vi "Host Image Acquisition Module.vi"(8 "error in":errorcluster, 11 "Operation":T3) -> (0 "error out":errorcluster, 1 "Image Acquired":bool, 2 "Acq In Progress":bool, 3 "Image":T2(plugin-control), 4 "Frames To Acquire":u32, 5 "Num Frames read":u32)   [LabVIEW 2013]
uses:
  Host Image Acquisition Module Enum.ctl
  Acquisition Settings Cluster.ctl
  Image Acquisition Settings FG Enum.ctl
  System Status/Status FG Enum.ctl
  Image Processing/Mask ROI FG Enum.ctl
  <vilib>/rvi/interface/common/niFpgaWaitOnOcc.vi
  <vilib>/FPGAPlugInAG/PCIe-1473R/niLvFpga_Reset_PCIe-1473R.vi
  <vilib>/Utility/error.llb/Error Cluster From Error Code.vi
  <vilib>/rvi/errors/niLvFpgaAdjustHostInterfaceError.vi
  <vilib>/FPGAPlugInAG/PCIe-1473R/niLvFpga_Run_PCIe-1473R.vi
  Globals/Average Sector Data.vi
  <vilib>/FPGAPlugInAG/PCIe-1473R/niLvFpga_Close_PCIe-1473R.vi
  <vilib>/rvi/interface/nirviMethod/nirviMethod.xnode
  FGs/FPGA_Reference.ctl
  FPGA Bitfiles/Simulation_WBA.lvbitx
  <vilib>/rvi/interface/nirviReadWriteControl/nirviReadWriteControl.xnode
  Common/CL Configuration.ctl
  Common/CL Signal Mapping.ctl
  FPGA/Sector/Accumulate/Sector Parameter Cluster.ctl
  <vilib>/rvi/interface/nirviCloseFPGA/nirviCloseFPGA.xnode
  Common/Timing/Timing Lib.lvlib
  NiFpgaLv.dll
  <vilib>/rvi/errors/niLvFpgaMergeErrorWithErrorCode.vi
  <vilib>/FPGAPlugInAG/PCIe-1473R/niLvFpga_ReadFifo_PCIe-1473R.vi
  <vilib>/FPGAPlugInAG/PCIe-1473R/niLvFpga_ConfigureFifo_PCIe-1473R.vi
  <vilib>/FPGAPlugInAG/PCIe-1473R/niLvFpga_StartFifo_PCIe-1473R.vi
panel:
  out "Actual Depth":u32
  out "Target Sim TO":bool
  out "Cam Data Timeout":bool
  out "Sector FIFO Timeout":bool
  out "Host DMA Timeout":bool
  out "Number of Elements to Write Host DMA":u32
  out "Number of Elements to Read Cam Data":u32
  out "Image Data":u64[](array[numeric])
  out "Elements Remaining":u32
  out "Words per image":u32
  out "DMA Words per Image":u32
  out "Acquire":bool
  in  "Acquisition Settings Cluster":T1={"Image Width"=1200, "Image Height"=788, "Frames To Acquire"=0, "Signal Mapping"=enum."Standard", "DMA Buffer Size\n(In Images)"=2200} {"Image Height" max=65535; "Image Width" max=65535 step=40}
  out "Buffer Size":u32
  out "Acq'd Frame Width":u32=2040
  out "DMA Write Timeout":bool
  in  "Start Serial Server":bool
  out "Frames Acq'd":u32=1
  out "Acq'd Frame Height":u32=1088
  out "Initialized":bool
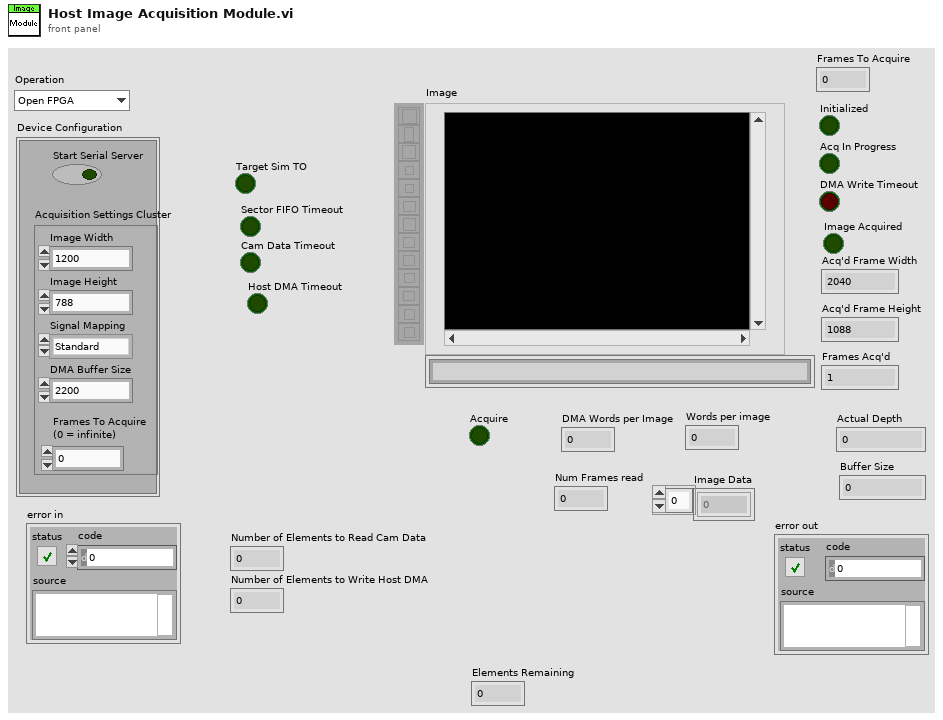
[diagram p1: front panel]
types:
  T1 = typedef "Acquisition Settings Cluster.ctl" = cluster{"Image Width":u32, "Image Height":u32, "Frames To Acquire":u32, "Signal Mapping":enum8{"Standard", "Basler 10-tap", "Vosskühler 10-tap"}, "DMA Buffer Size\n(In Images)":u32}
  T2 = typedef "IMAQ Image.ctl" = refnum<image>
  T3 = typedef "Host Image Acquisition Module Enum.ctl" = enum16{"Open FPGA", "Initialize DMA FIFO", "Load Sim Images", "Initialize Acquisition", "Update Sector Parameters", "Start Acquisition", "Aquire Image", "Read Averages", "Cancel Acquisition", "Close FPGA"}
  T4 = enum8{"Standard", "Basler 10-tap", "Vosskühler 10-tap"}
  T5 = typedef "Image Acquisition Settings FG Enum.ctl" = enum16{"Read", "Write"}
  T6 = typedef "Status FG Enum.ctl" = enum16{"Reset", "Read", "Write"}
  T7 = typedef "Mask ROI FG Enum.ctl" = enum16{"Read", "Write", "Enable Background", "Disable Background"}
  T8 = enum16{"big-endian, network order", "native, host order", "little-endian"}
  T9 = typedef "FPGA_Reference.ctl" = refnum<k20>
  T10 = typedef "Mask ROI Cluster.ctl" = cluster{"left annulus":T11, "right annulus":T11, "Threshold Range":cluster{"Lower value":dbl, "Upper value":dbl}, "[Avg BG]":u8[], "Number of Sectors":u8, "Left ROI":T12, "Right ROI":T12, "Left Start Angle Duty Cycle":fxp<+,8,0>, "Left End Angle Duty Cycle":fxp<+,8,0>, "Right End Angle Duty Cycle":fxp<+,8,0>, "Right Start Angle Duty Cycle":fxp<+,8,0>, "[Sector ROIs]":T12[]}
  T11 = typedef "IMAQ Circle" = cluster{"Center X":i32, "Center Y":i32, "Inner Radius":i32, "Outer Radius":i32, "Start Angle":dbl, "End Angle":dbl}
  T12 = typedef "ROI Descriptor" = cluster{"Global Rectangle":i32[], "Contours":cluster{"ID":enum32{"External", "Internal"}, "Type":u32, "Coordinates":i32[]}[]}
  T13 = typedef "Sector Parameter Cluster.ctl" = cluster{"Start Angle":fxp<+/-,17,2>, "End Angle":fxp<+/-,17,2>, "Inner Radius":u16, "Outter Radius":u16, "Hinge X":u16, "Hinge Y":u16, "NumWingSectors":u8}
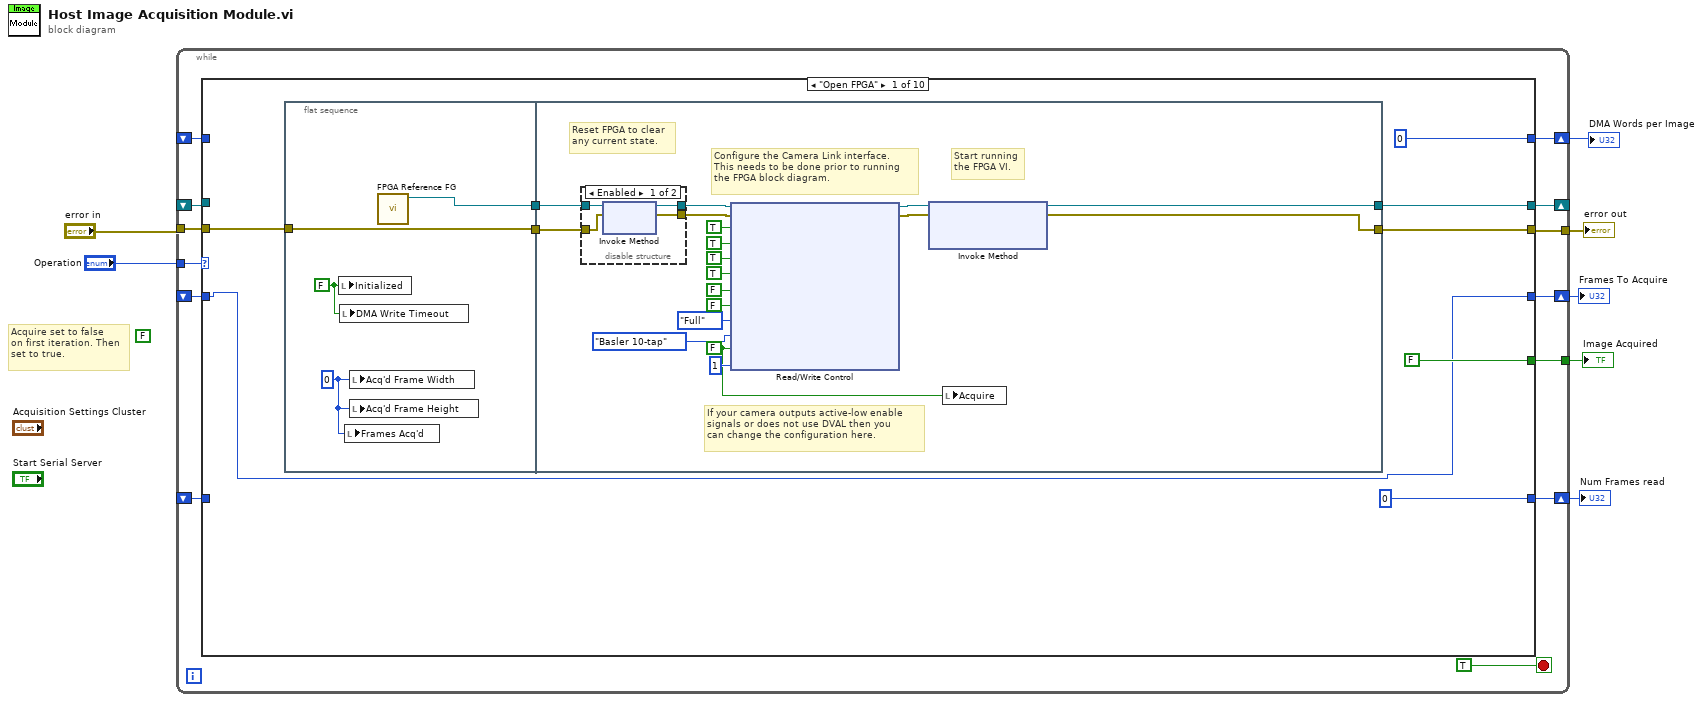
[diagram p0: block diagram]
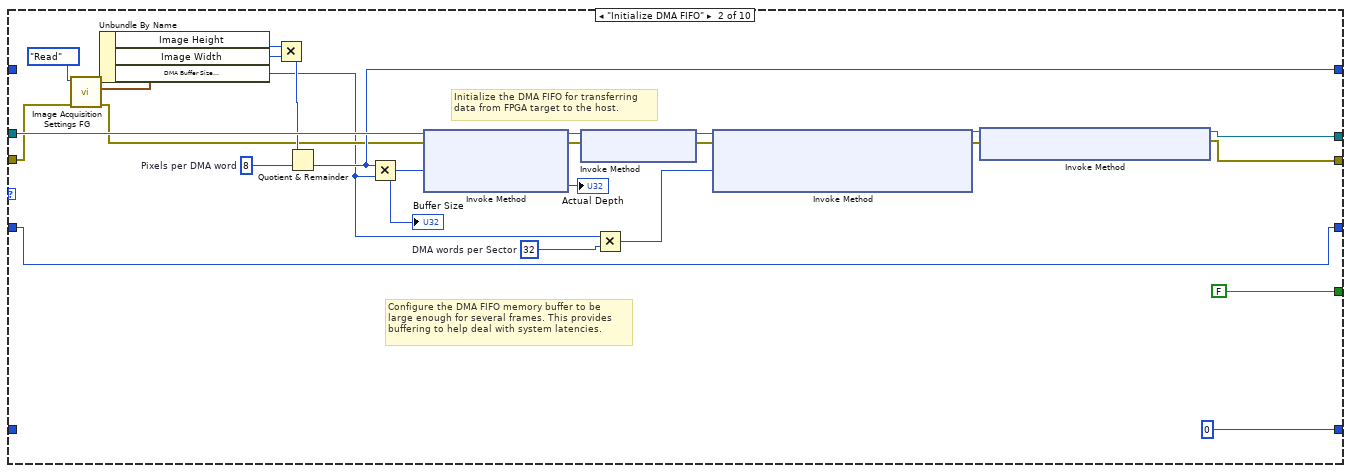
[diagram p3: hidden frame]
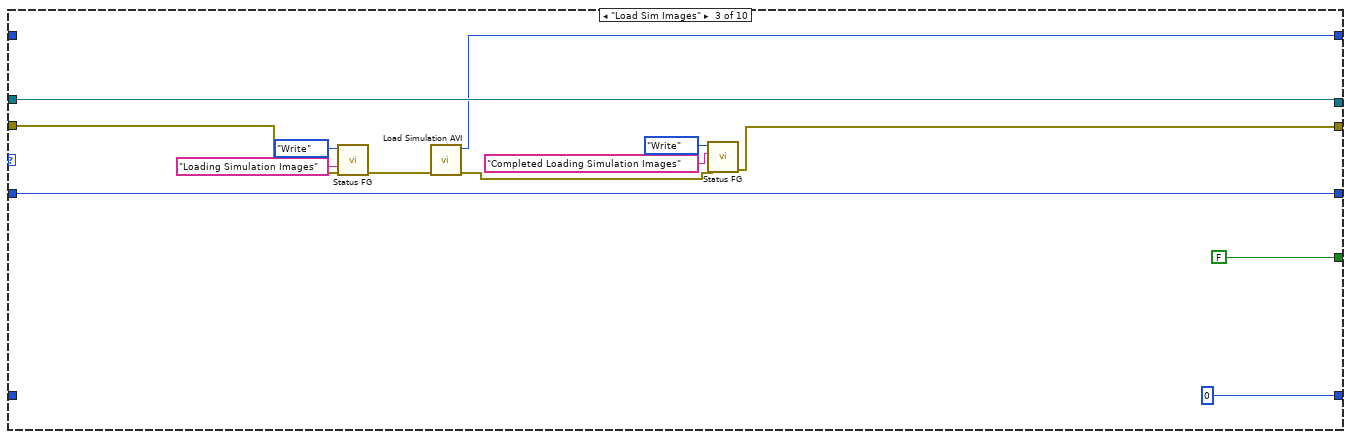
[diagram p4: hidden frame]
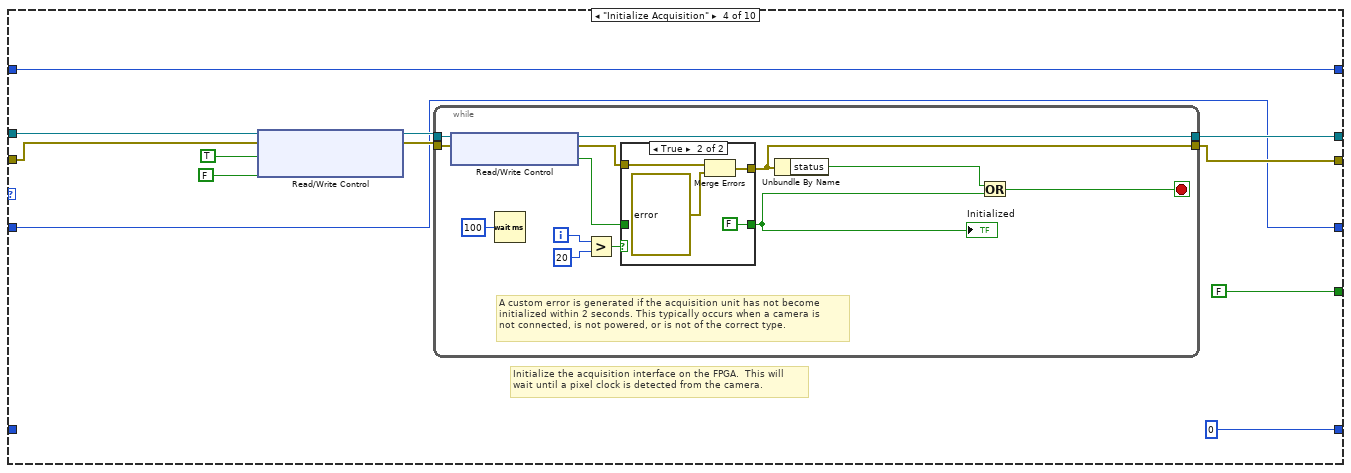
[diagram p5: hidden frame]
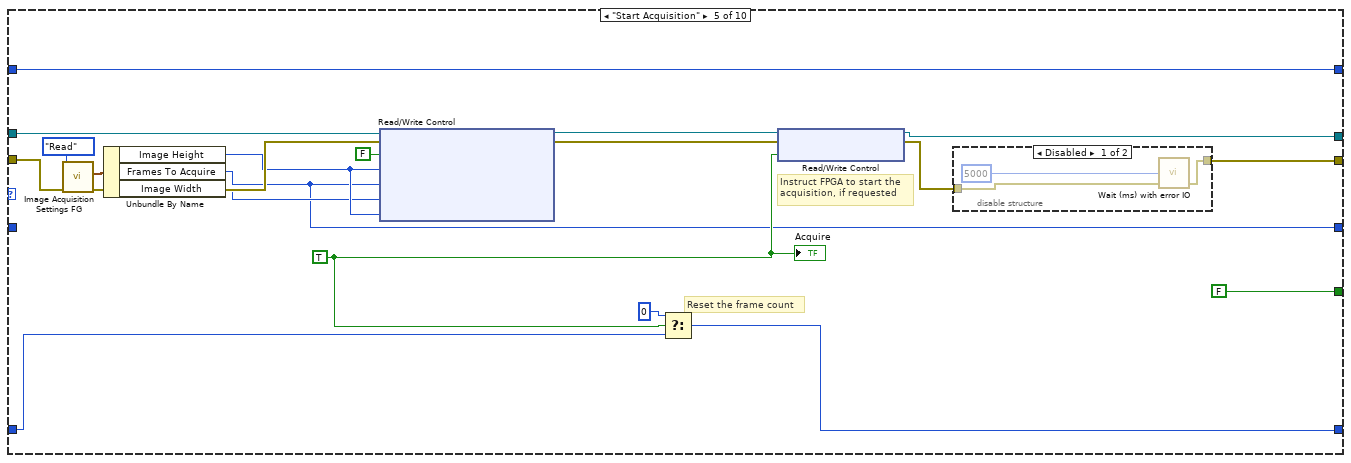
[diagram p7: hidden frame]
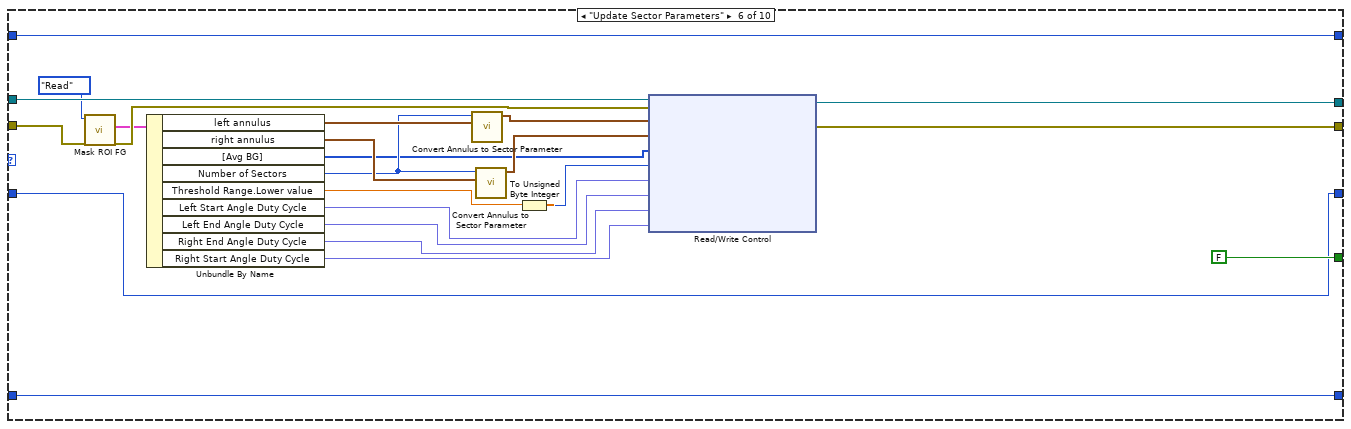
[diagram p9: hidden frame]
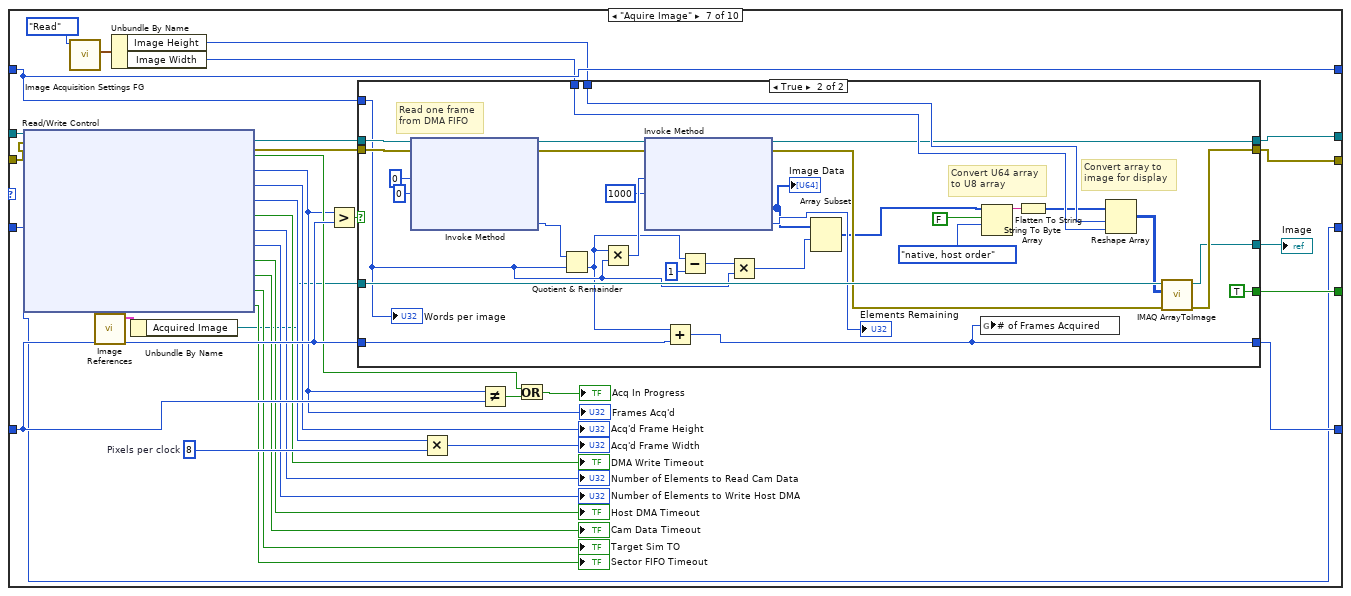
[diagram p10: hidden frame]
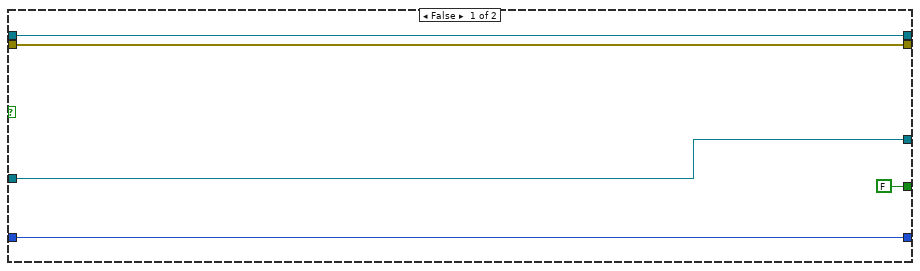
[diagram p11: hidden frame]
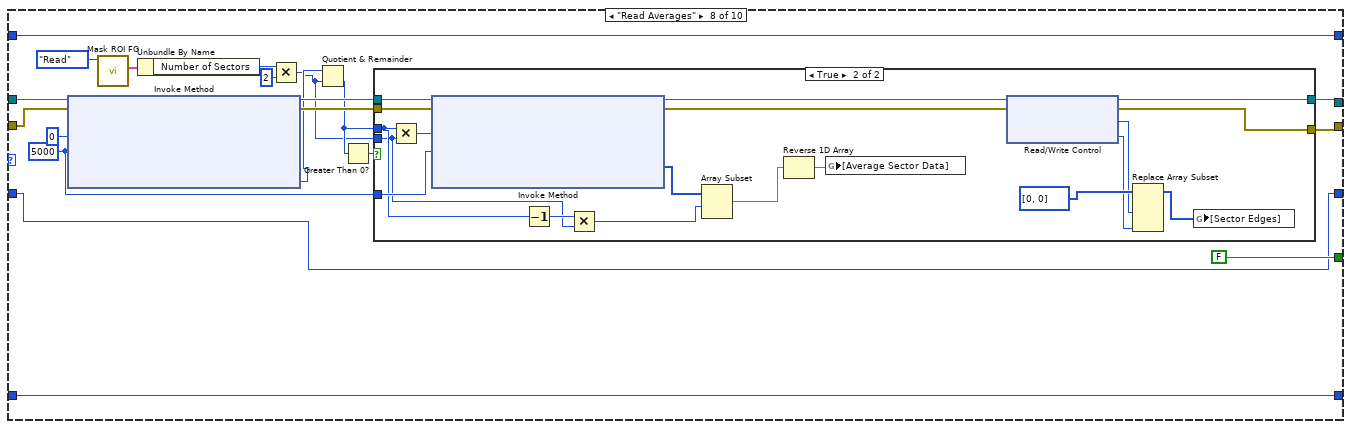
[diagram p12: hidden frame]
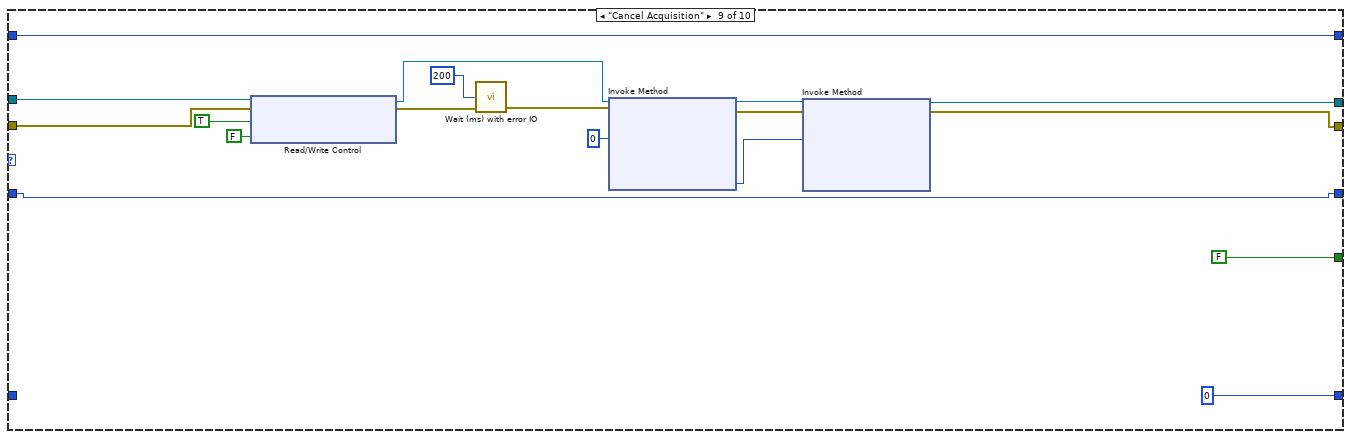
[diagram p14: hidden frame]
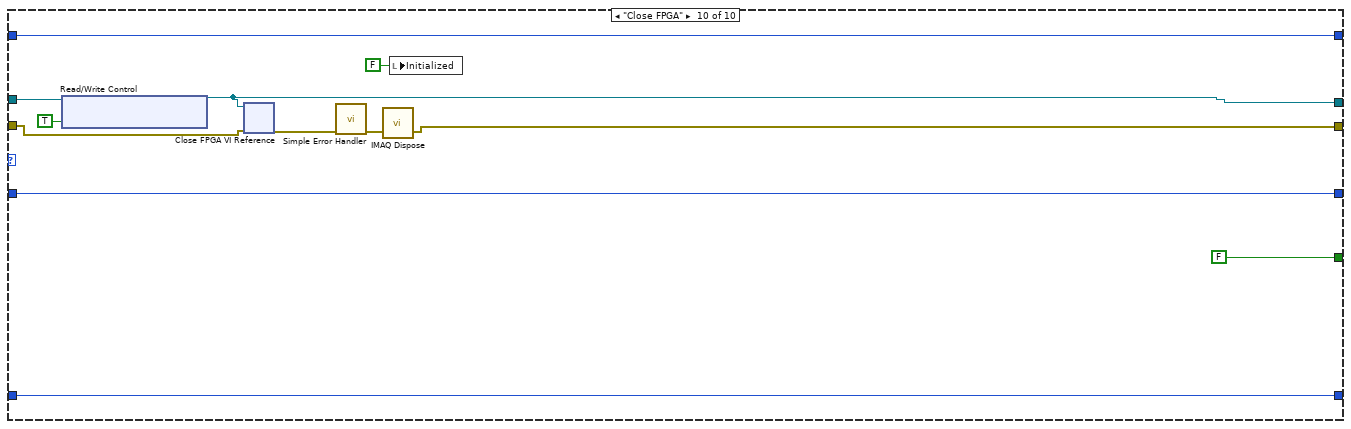
[diagram p15: hidden frame]
diagram:
  (unwired) FALSE ("Acquire")
  # "Acquire set to false\non first iteration. Then\nset to true."
  n1 = while {
    shift-right: [w19] -> _
    shift-left: _ -> [w15]
    tunnel: "error in" -> [w18]
    tunnel: "Operation" -> [w17]
    tunnel: [w16] -> w5
    shift-right: [w14] -> w4
    shift-left: _ -> [w13]
    shift-right: [w12] -> w3
    shift-left: _ -> [w11]
    tunnel: [w10] -> w2
    shift-right: [w9] -> w1
    shift-left: _ -> [w8]
    stop <- TRUE stop-if-true
    n2 = case shown="\"Open FPGA\"" w17 {
      tunnel: w18 -> [w29 w80 w92 w103 w146 w172 w203 w259 w303 w311]
      tunnel: [w28 w79 w95 w107 w142 w170 w207 w264 w289 w312] -> w19
      tunnel: [w27 w59 w91 w104 w141 w171 w206 w260 w288 w316] -> w16
      tunnel: w15 -> [_ w83 w95 w108 w147 w174 w208 w265 w304 w313]
      tunnel: [u32 0 w82 w94 w106 w143 w173 w204 w263 w302 w314] -> w14
      tunnel: w13 -> [_ _ _ w106 w143 w173 w204 w263 w302 w314]
      tunnel: [u32 0 u32 0 u32 0 u32 0 w144 w169 w205 w262 u32 0 w315] -> w12
      tunnel: w11 -> [_ _ _ _ w145 w169 w202 w262 _ w315]
      tunnel: [FALSE ("Image Acquired") FALSE ("Image Acquired") FALSE ("Image Acquired") FALSE ("Image Acquired") FALSE ("Image Acquired") FALSE ("Image Acquired") w201 FALSE ("Image Acquired") FALSE ("Image Acquired") FALSE ("Image Acquired")] -> w10
      tunnel: [w21 w58 w84 w97 w128 w152 w175 w246 w287 w305] -> w9
      tunnel: w8 -> [w21 w58 w84 w97 _ w152 w175 w246 w287 w305]
      frame "Open FPGA" {
        n3 = flat-sequence {
          tunnel: w29 -> [w30]
          tunnel: [w31] -> w26
          tunnel: [w30] -> w25
          tunnel: [w48] -> w27
          tunnel: [w49] -> w28
          tunnel: w26 -> [w51]
          tunnel: w25 -> [w50]
          frame #0 {
            w32 = u32 0 ("Acq'd Frame Width")
            w33 = FALSE ("Initialized")
            n4 = local write "Initialized"(w33) -> ()
            n5 = local write "DMA Write Timeout"(w33) -> ()
            n6 = local write "Frames Acq'd"(w32) -> ()
            n7 = local write "Acq'd Frame Width"(w32) -> ()
            n8 = local write "Acq'd Frame Height"(w32) -> ()
            n9 = call "FPGA Reference FG.vi"() -> ("FPGA VI Reference Out"=w31:T9)  [unwired: 11 in]
          }
          frame #1 {
            w34 = FALSE ("Acq Control.Acquire")
            # "If your camera outputs active-low enable\nsignals or does not use DVAL then you \ncan change the configuration here."
            # "Start running\nthe FPGA VI."
            # "Reset FPGA to clear\nany current state."
            # "Configure the Camera Link interface.\nThis needs to be done prior to running\nthe FPGA block diagram."
            n10 = disable-structure shown="Enabled" {
              disable-tunnel: [w55 w57] -> w41
              disable-tunnel: [w54 w56] -> w39
              disable-tunnel: w51 -> [w53 w57]
              disable-tunnel: w50 -> [w52 w56]
              frame Enabled {
                n11 = xnode "Invoke Method"("FPGA VI Reference In"=w53, "error in"=w52) -> ("FPGA VI Reference Out"=w55:T9, "error out"=w54:errorcluster)
              }
              frame Disabled {
              }
            }
            n12 = xnode "Read/Write Control"("FPGA VI Reference In"=w41, "error in"=w39, "CL Config.FVAL Active High"=TRUE ("IO Module Config.CL FVAL Active High"), "CL Config.LVAL Active High"=TRUE ("IO Module Config.CL LVAL Active High"), "CL Config.DVAL Active High"=TRUE ("IO Module Config.CL DVAL Active High"), "CL Config.Spare Active High"=TRUE ("IO Module Config.CL Spare Active High"), "CL Config.Line Scan"=FALSE, "Acq Control.Ignore DVAL"=FALSE ("CL Config.Line Scan"), "CL Config.Configuration"=enum8{"Base", "Medium", "Full"}."Full", "CL Config.Signal Mapping"=T4."Basler 10-tap", "Acq Control.Acquire"=w34, "# of Frames to Average"=u8 1) -> ("FPGA VI Reference Out"=w38:T9, "error out"=w40:errorcluster)
            n13 = xnode "Invoke Method"("FPGA VI Reference In"=w38, "error in"=w40) -> ("FPGA VI Reference Out"=w49:T9, "error out"=w48:errorcluster)  [unwired: 1 in]
            n14 = local write "Acquire"(w34) -> ()
          }
        }
      }
      frame "Initialize DMA FIFO" {
        w62 = u32 32  # DMA words per Sector
        w74 = u32 8  # Pixels per DMA word
        # "Configure the DMA FIFO memory buffer to be\nlarge enough for several frames. This provides\nbuffering to help deal with system latencies."
        # "Initialize the DMA FIFO for transferring\ndata from FPGA target to the host."
        n15 = call "Image Acquisition Settings FG.vi"("error in (no error)"=w80, "Operation"=Image_Acquisition_Settings_FG_Enum."Read") -> ("error out"=w68:errorcluster, "Acquisition Settings Out"=w71:T1)  [unwired: 8 in]
        n16 = Unbundle By Name(w71) -> ("Image Height"=w70:u32, "Image Width"=w69:u32, "DMA Buffer Size\n(In Images)"=w61:u32)
        n17 = Multiply(x=w70, y=w69) -> (x*y=w73:u32)
        n18 = Quotient & Remainder(x=w73, y=w74) -> (floor(x/y)=w82:u32)  [unwired: 1 out]
        n19 = Multiply(x=w82, y=w61) -> (x*y=w75:u32)
        "Buffer Size" <- w75
        n20 = xnode "Invoke Method"("FPGA VI Reference In"=w83, "error in"=w68, "Requested Depth"=w75) -> ("FPGA VI Reference Out"=w77:T9, "error out"=w76:errorcluster, "Actual Depth"=→"Actual Depth":u32)
        n21 = xnode "Invoke Method"("FPGA VI Reference In"=w77, "error in"=w76) -> ("FPGA VI Reference Out"=w67:T9, "error out"=w65:errorcluster)
        n22 = Multiply(x=w61, y=w62) -> (x*y=w60:u32)
        n23 = xnode "Invoke Method"("FPGA VI Reference In"=w67, "error in"=w65, "Requested Depth"=w60) -> ("FPGA VI Reference Out"=w64:T9, "error out"=w63:errorcluster)  [unwired: 1 out]
        n24 = xnode "Invoke Method"("FPGA VI Reference In"=w64, "error in"=w63) -> ("FPGA VI Reference Out"=w79:T9, "error out"=w59:errorcluster)
      }
      frame "Load Sim Images" {
        n25 = call "Status FG.vi"("error in (no error)"=w92, "Status In"="Loading Simulation Images", "Operation"=Status_FG_Enum."Write") -> ("error out"=w90:errorcluster)  [unwired: 7 in, 1 out]
        n26 = call "Load Simulation AVI.vi"("error in (no error)"=w90) -> ("error out"=w86:errorcluster, "Words per image"=w94:u32)  [unwired: 9 in]
        n27 = call "Status FG.vi"("error in (no error)"=w86, "Status In"="Completed Loading Simulation Images", "Operation"=Status_FG_Enum."Write") -> ("error out"=w91:errorcluster)  [unwired: 7 in, 1 out]
      }
      frame "Initialize Acquisition" {
        # "Initialize the acquisition interface on the FPGA.  This will\nwait until a pixel clock is detected from the camera."
        n28 = xnode "Read/Write Control"("FPGA VI Reference In"=w108, "error in"=w103, "Acq Control.Initialize"=TRUE ("Arm Acquisition"), "Acq Control.Cancel Acq"=FALSE) -> ("FPGA VI Reference Out"=w101:T9, "error out"=w100:errorcluster)
        n29 = while {
          tunnel: w101 -> [w117]
          tunnel: w100 -> [w116]
          tunnel: [w115] -> w107
          tunnel: [w118] -> w104
          i -> [w111]
          stop <- w121 stop-if-true
          # "A custom error is generated if the acquisition unit has not become\ninitialized within 2 seconds. This typically occurs when a camera is\nnot connected, is not powered, or is not of the correct type."
          n30 = xnode "Read/Write Control"("FPGA VI Reference In"=w117, "error in"=w116) -> ("FPGA VI Reference Out"=w115:T9, "error out"=w114:errorcluster, "Acq Status.Initialized"=w113:bool)
          n31 = Wait (ms)(milliseconds to wait=u32 100) -> ()  [unwired: 1 out]
          n32 = Greater?(x=w111, y=20) -> (0:w112:bool)
          n33 = case shown="True" w112 {
            tunnel: [w123 FALSE] -> w109
            tunnel: w113 -> [w123 _]
            tunnel: w114 -> [w122 w125]
            tunnel: [w122 w127] -> w118
            frame False {
            }
            frame True {
              n34 = Merge Errors(w125, errorcluster {"status"=TRUE, "code"=-8999, "source"="Acquisition Initialization: This error typically occurs when a camera is not properly connected, is not powered, or is not of the correct type."} ("error in")) -> (w127:errorcluster)
            }
          }
          "Initialized" <- w109
          n35 = Unbundle By Name(w118) -> ("status"=w120:bool)
          n36 = Or(x=w120, y=w109) -> (x .or. y?=w121:bool)
        }
      }
      frame "Start Acquisition" {
        w136 = TRUE ("Acquire")
        # "Reset the frame count"
        # "Instruct FPGA to start the\nacquisition, if requested"
        n37 = call "Image Acquisition Settings FG.vi"("error in (no error)"=w146, "Operation"=Image_Acquisition_Settings_FG_Enum."Read") -> ("error out"=w135:errorcluster, "Acquisition Settings Out"=w139:T1)  [unwired: 8 in]
        n38 = Unbundle By Name(w139) -> ("Image Height"=w130:u32, "Frames To Acquire"=w128:u32, "Image Width"=w129:u32)
        n39 = xnode "Read/Write Control"("FPGA VI Reference In"=w147, "error in"=w135, "Acq Control.Cancel Acq"=FALSE, "Acq Control.Line Scan Height"=w130, "Acq Control.Frames To Acq"=w128, "X Resolution"=w129, "Y Resolution"=w130) -> ("FPGA VI Reference Out"=w131:T9, "error out"=w132:errorcluster)
        n40 = Select(t=u32 0, s=w136, f=w145) -> (s? t:f=w144:u32)
        n41 = xnode "Read/Write Control"("FPGA VI Reference In"=w131, "error in"=w132, "Acq Control.Acquire"=w136) -> ("FPGA VI Reference Out"=w142:T9, "error out"=w133:errorcluster)
        n42 = disable-structure shown="Disabled" {
          disable-tunnel: w133 -> [w149 w151]
          disable-tunnel: [w148 w151] -> w141
          frame Disabled {
            n43 = call "Wait (ms) with error IO.vi"("error in (no error)"=w149, "milliseconds to wait"=u32 5000) -> ("error out"=w148:errorcluster)  [unwired: 3 in]
          }
          frame Enabled {
          }
        }
        "Acquire" <- w136
      }
      frame "Update Sector Parameters" {
        n44 = call "Mask ROI FG.vi"("error in (no error)"=w172, "Operation"=Mask_ROI_FG_Enum."Read") -> ("error out"=w167:errorcluster, "Mask ROI Out"=w165:T10)  [unwired: 8 in]
        n45 = Unbundle By Name(w165) -> ("left annulus"=w164:T11, "right annulus"=w162:T11, "[Avg BG]"=w159:u8[], "Number of Sectors"=w161:u8, "Threshold Range.Lower value"=w158:dbl, "Left Start Angle Duty Cycle"=w156:fxp<+,8,0>, "Left End Angle Duty Cycle"=w155:fxp<+,8,0>, "Right End Angle Duty Cycle"=w154:fxp<+,8,0>, "Right Start Angle Duty Cycle"=w153:fxp<+,8,0>)
        n46 = call "Convert Annulus to Sector Parameter.vi"("Annulus"=w164, "NumWingSectors"=w161) -> ("Sector Parameter"=w163:T13)  [unwired: 9 in]
        n47 = call "Convert Annulus to Sector Parameter.vi"("Annulus"=w162, "NumWingSectors"=w161) -> ("Sector Parameter"=w160:T13)  [unwired: 9 in]
        n48 = To Unsigned Byte Integer(number=w158) -> (unsigned 8bit integer=w157:u8)
        n49 = xnode "Read/Write Control"("FPGA VI Reference In"=w174, "error in"=w167, "Sector Parameters Left"=w163, "Sector Parameters Right"=w160, "[Average BG Intensity]"=w159, "Sector Threshold"=w157, "Left Start Angle Duty Cycle"=w156, "Left End Angle Duty Cycle"=w155, "Right End Angle Duty Cycle"=w154, "Right Start Angle Duty Cycle"=w153) -> ("FPGA VI Reference Out"=w170:T9, "error out"=w171:errorcluster)
      }
      frame "Aquire Image" {
        w196 = u32 8  # Pixels per clock
        n50 = xnode "Read/Write Control"("FPGA VI Reference In"=w208, "error in"=w203) -> ("FPGA VI Reference Out"=w200:T9, "error out"=w199:errorcluster, "Acq Status.Acq In Progress"=w188:bool, "Acq Status.Frames Acq'd"=w187:u32, "Acq Status.Lines Per Frame"=→"Acq'd Frame Height":u32, "Acq Status.Clocks Per Line"=w195:u32, "Acq Status.DMA Write Timeout"=→"DMA Write Timeout":bool, "Number of Elements to Read Cam Data"=→"Number of Elements to Read Cam Data":u32, "Number of Elements to Write Host DMA"=→"Number of Elements to Write Host DMA":u32, "Host DMA Timeout"=→"Host DMA Timeout":bool, "Cam Data Timeout"=→"Cam Data Timeout":bool, "Target Sim TO"=→"Target Sim TO":bool, "Sector FIFO Timeout"=→"Sector FIFO Timeout":bool)
        "Frames Acq'd" <- w187
        n51 = call "Image Acquisition Settings FG.vi"("Operation"=Image_Acquisition_Settings_FG_Enum."Read") -> ("Acquisition Settings Out"=w191:T1)  [unwired: 9 in, 1 out]
        n52 = call "Image References.vi"() -> ("Images"=w178:cluster{"Acquired Image":T2, "Display Image":T2})  [unwired: 10 in, 1 out]
        n53 = Unbundle By Name(w191) -> ("Image Height"=w190:u32, "Image Width"=w189:u32)
        n54 = Unbundle By Name(w178) -> ("Acquired Image"=w177:T2)
        n55 = Greater?(x=w187, y=w202) -> (0:w198:bool)
        n56 = case shown="True" w198 {
          tunnel: w200 -> [w212 w238]
          tunnel: w199 -> [w211 w239]
          tunnel: w190 -> [_ w245]
          tunnel: w189 -> [_ w244]
          tunnel: w177 -> [w213 w243]
          tunnel: [w211 w242] -> w206
          tunnel: [w212 w220] -> w207
          tunnel: w202 -> [w210 w217]
          tunnel: [w210 w215] -> w205
          tunnel: w204 -> [_ w223]
          tunnel: [w213 w241] -> w176
          tunnel: [FALSE ("Image Acquired") TRUE ("Image Acquired")] -> w201
          frame False {
          }
          frame True {
            # "Convert U64 array\nto U8 array"
            # "Convert array to\nimage for display"
            # "Read one frame\nfrom DMA FIFO"
            n57 = xnode "Invoke Method"("FPGA VI Reference In"=w238, "error in"=w239, "Number of Elements"=u32 0, "Timeout (ms)"=0) -> ("FPGA VI Reference Out"=w229:T9, "error out"=w228:errorcluster, "Elements Remaining"=w230:u32)  [unwired: 1 out]
            n58 = Quotient & Remainder(x=w230, y=w223) -> (floor(x/y)=w218:u32)  [unwired: 1 out]
            n59 = Multiply(x=w218, y=w223) -> (x*y=w227:u32)
            n60 = xnode "Invoke Method"("FPGA VI Reference In"=w229, "error in"=w228, "Number of Elements"=w227, "Timeout (ms)"=1000) -> ("FPGA VI Reference Out"=w220:T9, "error out"=w219:errorcluster, "Data"=w216:u64[], "Elements Remaining"=→"Elements Remaining":u32)
            "Image Data" <- w216
            n61 = Add(x=w218, y=w217) -> (x+y=w215:u32)
            n62 = Subtract(x=w218, y=u32 1) -> (x-y=w224:u32)
            n63 = Multiply(x=w224, y=w223) -> (x*y=w222:u32)
            n64 = Array Subset(array=w216, index=w222) -> (w214:u64[])  [unwired: 1 in]
            n65 = global write "Average Sector Data.vi" "# of Frames Acquired"(w215) -> ()
            n66 = Flatten To String(anything=w214, prepend array or string size? (T)=FALSE, byte order (0:big-endian, network order)=T8."native, host order") -> (data string=w232:string)  [unwired: 1 in, 2 out]
            n67 = String To Byte Array(string=w232) -> (unsigned byte array=w231:u8[])
            n68 = Reshape Array(w231, w245, w244) -> (w235:u8[][])
            n69 = call "IMAQ ArrayToImage"("error in (no error)"=w219, "Image Pixels (U8)"=w235, "Image"=w243) -> ("error out"=w242:errorcluster, "Image Out"=w241:T2)  [unwired: 7 in]
            "Words per image" <- w223
          }
        }
        "Image" <- w176
        n70 = Multiply(x=w195, y=w196) -> (x*y=→"Acq'd Frame Width":u32)
        n71 = Not Equal?(x=w187, y=w202) -> (x != y?=w186:bool)
        n72 = Or(x=w188, y=w186) -> (x .or. y?=→"Acq In Progress":bool)
      }
      frame "Read Averages" {
        w255 = 5000 ("Timeout (ms)")
        n73 = xnode "Invoke Method"("FPGA VI Reference In"=w265, "error in"=w259, "Number of Elements"=u32 0, "Timeout (ms)"=w255) -> ("FPGA VI Reference Out"=w257:T9, "error out"=w256:errorcluster, "Elements Remaining"=w249:u32)  [unwired: 1 out]
        n74 = call "Mask ROI FG.vi"("Operation"=Mask_ROI_FG_Enum."Read") -> ("Mask ROI Out"=w253:T10)  [unwired: 9 in, 1 out]
        n75 = Unbundle By Name(w253) -> ("Number of Sectors"=w251:u8)
        n76 = Multiply(x=w251, y=u8 2) -> (x*y=w247:u8)
        n77 = Quotient & Remainder(x=w249, y=w247) -> (floor(x/y)=w248:u32)  [unwired: 1 out]
        n78 = Greater Than 0?(x=w248) -> (x > 0?=w252:bool)
        n79 = case shown="True" w252 {
          tunnel: w257 -> [w267 w286]
          tunnel: w256 -> [w266 w285]
          tunnel: w255 -> [_ w284]
          tunnel: [w267 w280] -> w264
          tunnel: [w266 w281] -> w260
          tunnel: w248 -> [_ w272]
          tunnel: w247 -> [_ w271]
          frame False {
          }
          frame True {
            n80 = Multiply(x=w272, y=w271) -> (x*y=w274:u32)
            n81 = xnode "Invoke Method"("FPGA VI Reference In"=w286, "error in"=w285, "Number of Elements"=w274, "Timeout (ms)"=w284) -> ("FPGA VI Reference Out"=w283:T9, "error out"=w282:errorcluster, "Data"=w270:u8[])  [unwired: 1 out]
            n82 = Decrement(x=w272) -> (x-1=w273:u32)
            n83 = Multiply(x=w273, y=w271) -> (x*y=w269:u32)
            n84 = Array Subset(array=w270, index=w269) -> (w268:u8[])  [unwired: 1 in]
            n85 = Reverse 1D Array(array=w268) -> (reversed array=w279:u8[])
            n86 = global write "Average Sector Data.vi" "[Average Sector Data]"(w279) -> ()
            n87 = xnode "Read/Write Control"("FPGA VI Reference In"=w283, "error in"=w282) -> ("FPGA VI Reference Out"=w280:T9, "error out"=w281:errorcluster, "Right Sector Edge"=w277:u8, "Left Sector Edge"=w276:u8)
            n88 = Replace Array Subset(array=u8[] [0, 0] ("[Sector Edges]"), new element #1=w277, new element #2=w276) -> (w275:u8[])  [unwired: 2 in]
            n89 = global write "Average Sector Data.vi" "[Sector Edges]"(w275) -> ()
          }
        }
      }
      frame "Cancel Acquisition" {
        n90 = xnode "Read/Write Control"("FPGA VI Reference In"=w304, "error in"=w303, "Acq Control.Cancel Acq"=TRUE, "Acq Control.Acquire"=FALSE) -> ("FPGA VI Reference Out"=w294:T9, "error out"=w297:errorcluster)
        n91 = call "Wait (ms) with error IO.vi"("error in (no error)"=w297, "milliseconds to wait"=u32 200) -> ("error out"=w295:errorcluster)  [unwired: 3 in]
        n92 = xnode "Invoke Method"("FPGA VI Reference In"=w294, "error in"=w295, "Number of Elements"=u32 0) -> ("FPGA VI Reference Out"=w292:T9, "error out"=w291:errorcluster, "Elements Remaining"=w290:u32)  [unwired: 1 in, 1 out]
        n93 = xnode "Invoke Method"("FPGA VI Reference In"=w292, "error in"=w291, "Number of Elements"=w290) -> ("FPGA VI Reference Out"=w289:T9, "error out"=w288:errorcluster)  [unwired: 1 in, 2 out]
      }
      frame "Close FPGA" {
        n94 = xnode "Read/Write Control"("FPGA VI Reference In"=w313, "Acq Control.Cancel Acq"=TRUE) -> ("FPGA VI Reference Out"=w312:T9)  [unwired: 1 in, 1 out]
        n95 = xnode "Close FPGA VI Reference"("FPGA VI Reference In"=w312, "error in"=w311) -> ("error out"=w309:errorcluster)
        n96 = call <vilib>:"Simple Error Handler.vi"("error in (no error)"=w309) -> ("error out"=w307:errorcluster)  [unwired: 4 in, 4 out]
        n97 = call "IMAQ Dispose"("error in (no error)"=w307) -> ("error out"=w316:errorcluster)  [unwired: 5 in]
        n98 = local write "Initialized"(FALSE ("Initialized")) -> ()
      }
    }
  }
  "error out" <- w5
  "DMA Words per Image" <- w4
  "Num Frames read" <- w3
  "Image Acquired" <- w2
  "Frames To Acquire" <- w1
